vi "Read Data and Draw to LV Picture.vi"(6 "Pixel Format":string, 7 "Picture Ref":refnum<vi>, 8 "error in (no error)":errorcluster, 11 "Buffer in":refnum<class "Buffer.lvclass">) -> (0 "error out":errorcluster, 2 "Picture":picture, 3 "Buffer out":refnum<class "Buffer.lvclass">)   [LabVIEW 2020]
uses:
  g_industrial_cam/Buffer/Buffer.lvclass
  g_industrial_cam/Buffer/Buffer.lvclass/Buffer.ctl
  g_industrial_cam/Buffer/DrawToPictureCore.vi
  g_industrial_cam/Buffer/Draw RGB8 to Picture.vi
  g_industrial_cam/Buffer/Draw Mono10 to Picture.vi
  g_industrial_cam/Buffer/Draw BGR8 to Picture.vi
  g_industrial_cam/Buffer/Draw Mono8 to Picture.vi
  g_industrial_cam/Buffer/Draw Mono12 to Picture.vi
  g_industrial_cam/Buffer/Draw Mono14 to Picture.vi
  g_industrial_cam/Buffer/Draw Mono16 to Picture.vi
  g_industrial_cam/Buffer/Draw Mono10p to Picture.vi
  g_industrial_cam/Buffer/Draw Mono12p to Picture.vi
  g_industrial_cam/Buffer/Draw Mono14p to Picture.vi
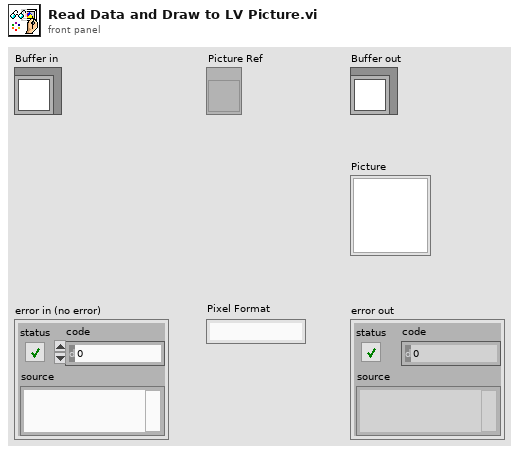
[diagram p1: front panel]
types:
  T1 = typedef "Buffer.lvclass/Image Size.ctl" = cluster{"Width":u16, "Height":u16}
  T2 = typedef "Buffer.lvclass/Picture Top Left Point Offset.ctl" = cluster{"x":i16, "y":i16}
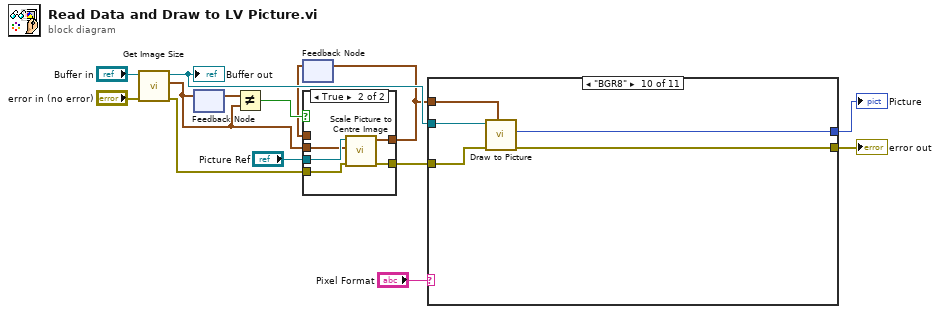
[diagram p0: block diagram]
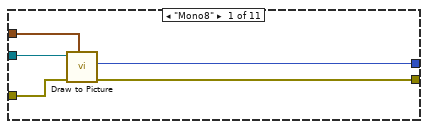
[diagram p3: hidden frame]
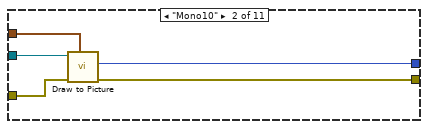
[diagram p4: hidden frame]
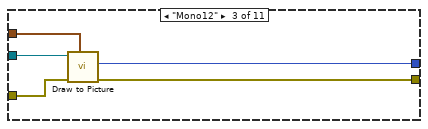
[diagram p5: hidden frame]
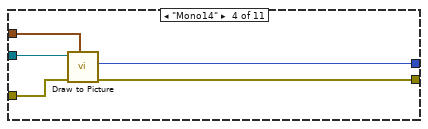
[diagram p6: hidden frame]
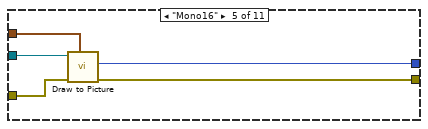
[diagram p7: hidden frame]
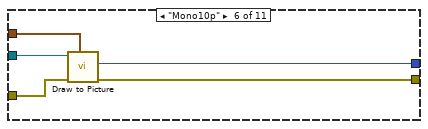
[diagram p8: hidden frame]
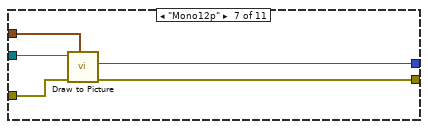
[diagram p9: hidden frame]
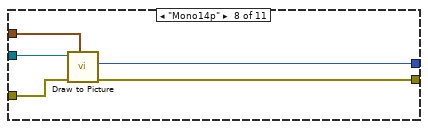
[diagram p10: hidden frame]
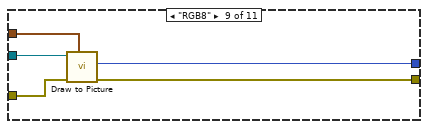
[diagram p11: hidden frame]
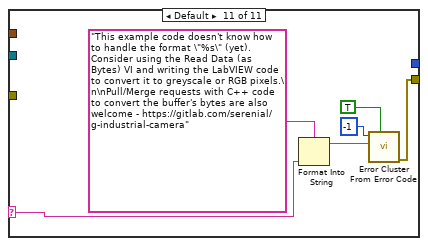
[diagram p12: hidden frame]
diagram:
  n1 = call "Get Image Size.vi"("error in (no error)"="error in (no error)", "Buffer in"="Buffer in") -> ("error out"=w7:errorcluster, "Image Size"=w4:T1, "Buffer"=w9:refnum<class "Buffer.lvclass">)  [unwired: 7 in]
  "Buffer out" <- w9
  n2 = feedback-in #1(w4) -> ()
  n3 = feedback #1() -> (w5:T1)  [unwired: 1 in]
  n4 = Not Equal?(x=w5, y=w4) -> (x != y?=w3:bool)
  n5 = feedback #2() -> (w1:T2)  [unwired: 1 in]
  n6 = case shown="True" w3 {
    tunnel: "Picture Ref" -> [_ w21]
    tunnel: w7 -> [w16 w20]
    tunnel: [w15 w19] -> w2
    tunnel: [w16 w18] -> w6
    tunnel: w4 -> [_ w17]
    tunnel: w1 -> [w15 _]
    frame False {
    }
    frame True {
      n7 = call "Scale Picture to Centre Image.vi"("error in (no error)"=w20, "Image Size"=w17, "Picture in"=w21) -> ("error out"=w18:errorcluster, "Draw Image to Picture Offset"=w19:T2)  [unwired: 6 in, 1 out]
    }
  }
  n8 = feedback-in #2(w2) -> ()
  n9 = case shown="\"BGR8\"" "Pixel Format" {
    selector: "Pixel Format" -> [_ _ _ _ _ _ _ _ _ _ w72]
    tunnel: w9 -> [w26 w31 w36 w41 w46 w51 w56 w61 w66 w71 _]
    tunnel: [w25 w30 w35 w40 w45 w50 w55 w60 w65 w69 w73] -> w13
    tunnel: [w24 w29 w34 w39 w44 w49 w54 w59 w64 w70 _] -> w14
    tunnel: w2 -> [w23 w28 w33 w37 w42 w48 w53 w58 w63 w68 _]
    tunnel: w6 -> [w22 w27 w32 w38 w43 w47 w52 w57 w62 w67 _]
    frame "Mono8" {
      n10 = call-poly "Draw to Picture.vi"("Top Left Point (0,0)"=w23, "error in (no error)"=w22, "Buffer in"=w26) -> ("error out"=w25:errorcluster, "Picture"=w24:picture)  [unwired: 6 in, 1 out]
    }
    frame "Mono10" {
      n11 = call-poly "Draw to Picture.vi"("Top Left Point (0,0)"=w28, "error in (no error)"=w27, "Buffer in"=w31) -> ("error out"=w30:errorcluster, "Picture"=w29:picture)  [unwired: 6 in, 1 out]
    }
    frame "Mono12" {
      n12 = call-poly "Draw to Picture.vi"("Top Left Point (0,0)"=w33, "error in (no error)"=w32, "Buffer in"=w36) -> ("error out"=w35:errorcluster, "Picture"=w34:picture)  [unwired: 6 in, 1 out]
    }
    frame "Mono14" {
      n13 = call-poly "Draw to Picture.vi"("Top Left Point (0,0)"=w37, "error in (no error)"=w38, "Buffer in"=w41) -> ("error out"=w40:errorcluster, "Picture"=w39:picture)  [unwired: 6 in, 1 out]
    }
    frame "Mono16" {
      n14 = call-poly "Draw to Picture.vi"("Top Left Point (0,0)"=w42, "error in (no error)"=w43, "Buffer in"=w46) -> ("error out"=w45:errorcluster, "Picture"=w44:picture)  [unwired: 6 in, 1 out]
    }
    frame "Mono10p" {
      n15 = call-poly "Draw to Picture.vi"("Top Left Point (0,0)"=w48, "error in (no error)"=w47, "Buffer in"=w51) -> ("error out"=w50:errorcluster, "Picture"=w49:picture)  [unwired: 6 in, 1 out]
    }
    frame "Mono12p" {
      n16 = call-poly "Draw to Picture.vi"("Top Left Point (0,0)"=w53, "error in (no error)"=w52, "Buffer in"=w56) -> ("error out"=w55:errorcluster, "Picture"=w54:picture)  [unwired: 6 in, 1 out]
    }
    frame "Mono14p" {
      n17 = call-poly "Draw to Picture.vi"("Top Left Point (0,0)"=w58, "error in (no error)"=w57, "Buffer in"=w61) -> ("error out"=w60:errorcluster, "Picture"=w59:picture)  [unwired: 6 in, 1 out]
    }
    frame "RGB8" {
      n18 = call-poly "Draw to Picture.vi"("Top Left Point (0,0)"=w63, "error in (no error)"=w62, "Buffer in"=w66) -> ("error out"=w65:errorcluster, "Picture"=w64:picture)  [unwired: 6 in, 1 out]
    }
    frame "BGR8" {
      n19 = call-poly "Draw to Picture.vi"("Top Left Point (0,0)"=w68, "error in (no error)"=w67, "Buffer in"=w71) -> ("error out"=w69:errorcluster, "Picture"=w70:picture)  [unwired: 6 in, 1 out]
    }
    frame Default {
      n20 = Format Into String(format string="This example code doesn't know how to handle the format \"%s\" (yet). Consider using the Read Data (as Bytes) VI and writing the LabVIEW code to convert it to greyscale or RGB pixels.\n\nPull/Merge requests with C++ code to convert the buffer's bytes are also welcome - https://gitlab.com/serenial/g-industrial-camera", w72) -> (resulting string=w77:string)  [unwired: 2 in, 1 out]
      n21 = call <vilib>:"Error Cluster From Error Code.vi"("show call chain? (False)"=TRUE, "error message (\"\")"=w77, "error code (0)"=-1) -> ("error out"=w73:errorcluster)  [unwired: 6 in]
    }
  }
  "error out" <- w13
  "Picture" <- w14
